vi "Ximea Camera Engine.vi"(0 "Ximea Notifier Name":string, 11 "Camera ID":string[](array[string])) -> ()   [LabVIEW 2016]
uses:
  Ximea Controls/Ximea ROI.ctl
  Ximea Controls/Ximea Parameters.ctl
  Ximea Controls/Ximea Parameter List.ctl
  xiLIB_64bit/xiLIB/xiCamLib/xiCam/PRM/PRM/PRM_v2.ctl
  Ximea Controls/Ximea Notifier Element.ctl
  Ximea Controls/Ximea Actions.ctl
  <vilib>/vision/Image Controls.llb/IMAQ Image.ctl
  Camera Controls/Camera IMAQ Key Info.ctl
panel:
  in  "Save Frames":bool
  in  "Use Display Module":bool
  in  "Quit":bool
  in  "Record":bool
  in  "Preview":bool
  out "Acquisition Loop":i32
  in  "Get Param":bool
  in  "Set Param":bool
  in  "Ximea  Parameter":T1
  in  "Get ROI":bool
  in  "Set ROI":bool
  in  "ROI Setup":T3
  out "Acquisition Frame":u32
  out "Serial No.":string
  out "Device Name":string
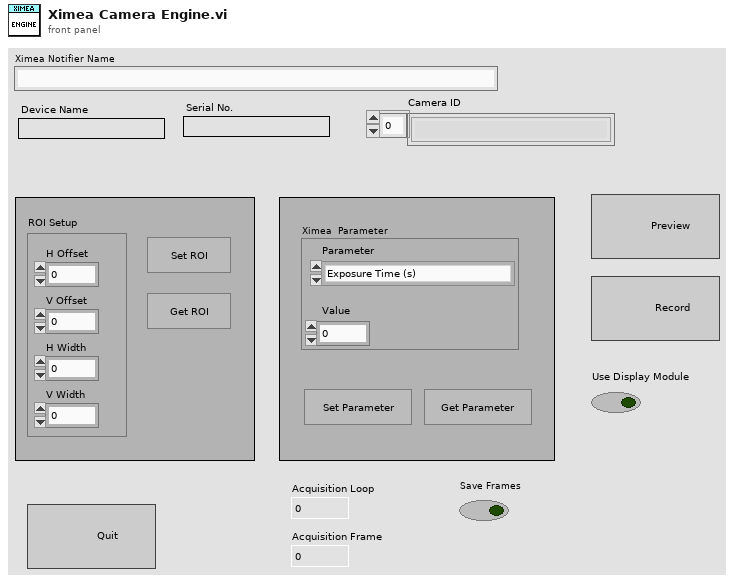
[diagram p1: front panel]
types:
  T1 = typedef "Ximea Parameters.ctl" = cluster{"Parameter":T2, "Value":sgl}
  T2 = typedef "Ximea Parameter List.ctl" = enum16{"Exposure Time (s)", "Gain"}
  T3 = typedef "Ximea ROI.ctl" = cluster{"H Offset":i32, "V Offset":i32, "H Width":i32, "V Width":i32}
  T4 = typedef "PRM_v2.ctl" = enum16{"ACQ_BUFFER_SIZE", "ACQ_FRAME_BURST_COUNT", "ACQ_TIMING_MODE", "ACQ_TRANSPORT_BUFFER_SIZE", "AE_MAX_LIMIT", "AEAG", "AEAG_LEVEL", "API_VERSION", "AG_MAX_LIMIT", "APPLY_CMS", "AUTO_BANDWIDTH_CALCULATION", "AUTO_WB", "AVAILABLE_BANDWIDTH", "AVAILABLE_BANDWIDTH_MAX", "AVAILABLE_BANDWIDTH_MIN", "BUFFER_POLICY", "BUFFERS_QUEUE_SIZE", "CC_MATRIX_00", "CC_MATRIX_01", "CC_MATRIX_02", "CC_MATRIX_03", "CC_MATRIX_10", "CC_MATRIX_11", "CC_MATRIX_12", "CC_MATRIX_13", "CC_MATRIX_20", "CC_MATRIX_21", "CC_MATRIX_22", "CC_MATRIX_23", "CC_MATRIX_30", "CC_MATRIX_31", "CC_MATRIX_32", "CC_MATRIX_33", "CHIP_TEMP", "CMS", "COLOR_FILTER_ARRAY", "COOLING", "DEBOUNCE_EN", "DEBOUNCE_POL", "DEBOUNCE_T0", "DEBOUNCE_T1", "DEBUG_LEVEL", "DEFAULT_CC_MATRIX", "DEVICE_INSTANCE_PATH", "DEVICE_MODEL_ID", "DEVICE_NAME", "DEVICE_SN", "DEVICE_TYPE", "DEVICE_USER_ID", "DOWNSAMPLING", "DOWNSAMPLING_TYPE", "DRV_VERSION", "EXP_PRIORITY", "EXPOSURE", "EXPOSURE_MAX", "EXPOSURE_MIN", "FFS_FILE_NAME", "FPGA1_VERSION", "FRAMERATE", "FRAMERATE_MAX", "FRAMERATE_MIN", "FREE_FFS_SIZE", "GAIN", "GAIN_MAX", "GAIN_MIN", "GAMMAC", "GAMMAY", "GPI_LEVEL", "GPI_MODE", "GPI_SELECTOR", "GPO_MODE", "GPO_SELECTOR", "HDR", "HDR_T1", "HDR_T2", "HEIGHT", "HEIGHT_MAX", "HEIGHT_MIN", "HOUSE_TEMP", "IMAGE_DATA_FORMAT", "IMAGE_IS_COLOR", "INPUT_CMS_PROFILE", "IS_COOLED", "IS_DEVICE_EXIST", "KNEEPOINT1", "KNEEPOINT2", "LED_MODE", "LED_SELECTOR", "LIMIT_BANDWIDTH", "LIMIT_BANDWIDTH_MAX", "LIMIT_BANDWIDTH_MIN", "LUT_EN", "LUT_INDEX", "LUT_INDEX_MAX", "LUT_INDEX_MIN", "LUT_VALUE", "LUT_VALUE_MAX", "LUT_VALUE_MIN", "MANUAL_WB", "MCU1_VERSION", "MCU2_VERSION", "OFFSET_X", "OFFSET_X_MAX", "OFFSET_X_MIN", "OFFSET_Y", "OFFSET_Y_MAX", "OFFSET_Y_MIN", "OUTPUT_CMS_PROFILE", "OUTPUT_DATA_BIT_DEPTH", "OUTPUT_DATA_PACKING", "READ_FILE_FFS", "RECENT_FRAME", "SENSOR_DATA_BIT_DEPTH", "SENSOR_MODE", "SENSOR_TAPS", "SHARPNESS", "SHUTTER_TYPE", "TARGET_TEMP", "TRG_DELAY", "TRG_SELECTOR", "TRG_SOFTWARE", "TRG_SOURCE", "USED_FFS_SIZE", "WB_KB", "WB_KG", "WB_KR", "WIDTH", "WIDTH_MAX", "WIDTH_MIN", "WRITE_FILE_FFS", "ACQ_BUFFER_SIZE_UNIT", "ACQ_TRANSPORT_BUFFER_COMMIT", "AEAG_ROI_HEIGHT", "AEAG_ROI_OFFSET_X", "AEAG_ROU_OFFSET_Y", "AEAG_ROI_WIDTH", "API_CONTEXT_LIST", "BINNING_HORIZONTAL", "BINNING_SELECTOR", "BINNING_VERTICAL", "COLUMN_FPN_CORRECTION", "COUNTER_SELECTOR", "COUNTER_VALUE", "DECIMATION_HORIZONTAL", "DECIMATION_SELECTOR", "DECIMATION_VERTICAL", "DEVICE_ID", "DEVICE_LOCATION_PATH", "DEVICE_MANIFEST", "DEVICE_RESET", "DEVICE_SENS_SN", "EXPOSURE_BURST_COUNT", "FFS_ACCESS_KEY", "GAIN_SELECTOR", "HW_REVISION", "IMAGE_BLACK_LEVEL", "IMAGE_DATA_BIT_DEPTH", "IMAGE_DATA_FORMAT_RGB32_ALPHA", "IMAGE_PAYLOAD_SIZE", "LENS_APERTURE_VALUE", "LENS_FEATURE", "LENS_FEATURE_SELECTOR", "LENS_FOCAL_LENGTH", "LENS_FOCUS_DISTANCE", "LENS_FOCUS_MOVE", "LENS_FOCUS_MOVEMENT_VALUE", "LENS_MODE", "OUTPUT_DATA_PACKING_TYPE", "SENSOR_CLOCK_FREQ_HZ", "SENSOR_CLOCK_FREQ_INDEX", "SENSOR_FEATURE_SELECTOR", "SENSOR_FEATURE_VALUE", "SENSOR_OUTPUT_CHANNEL_COUNT", "TRANSPORT_PIXEL_FORMAT", "TS_RST_MODE", "TS_RST_SOURCE", "SENS_DEFECTS_CORR_LIST_SELECTOR", "SENS_DEFECTS_CORR", "SENS_DEFECTS_CORR_LIST_CONTENT", "DEVICE_UNIT_SELECTOR", "DEVICE_UNIT_REGISTER_SELECTOR", "DEVICE_UNIT_REGISTER_VALUE"}
  T5 = typedef "Camera IMAQ Key Info.ctl" = cluster{"Frame":u32, "Sensor Height":i32, "Sensor Width":i32, "ROI Height":i32, "ROI Width":i32, "ROI Enable?":bool, "Bit per Pixel":u8}
  T6 = typedef "Image Type" = u32
  T7 = typedef "Ximea Notifier Element.ctl" = cluster{"Ximea Actions":T8, "Received?":bool, "Ximea Parameter":T1, "Ximea ROI":T3, "Running?":bool, "File Path":path, "# of frames":u32, "Image Ref":T9, "Error":errorcluster, "Trigger?":bool, "ROI Increment":i32}
  T8 = typedef "Ximea Actions.ctl" = enum16{"Idle", "Error Check", "Preview", "Record", "Soft Trigger", "Abort", "Record Settings", "Set Parameter", "Get Parameter", "Set ROI", "Get ROI", "Status", "Quit"}
  T9 = typedef "IMAQ Image.ctl" = refnum<image>
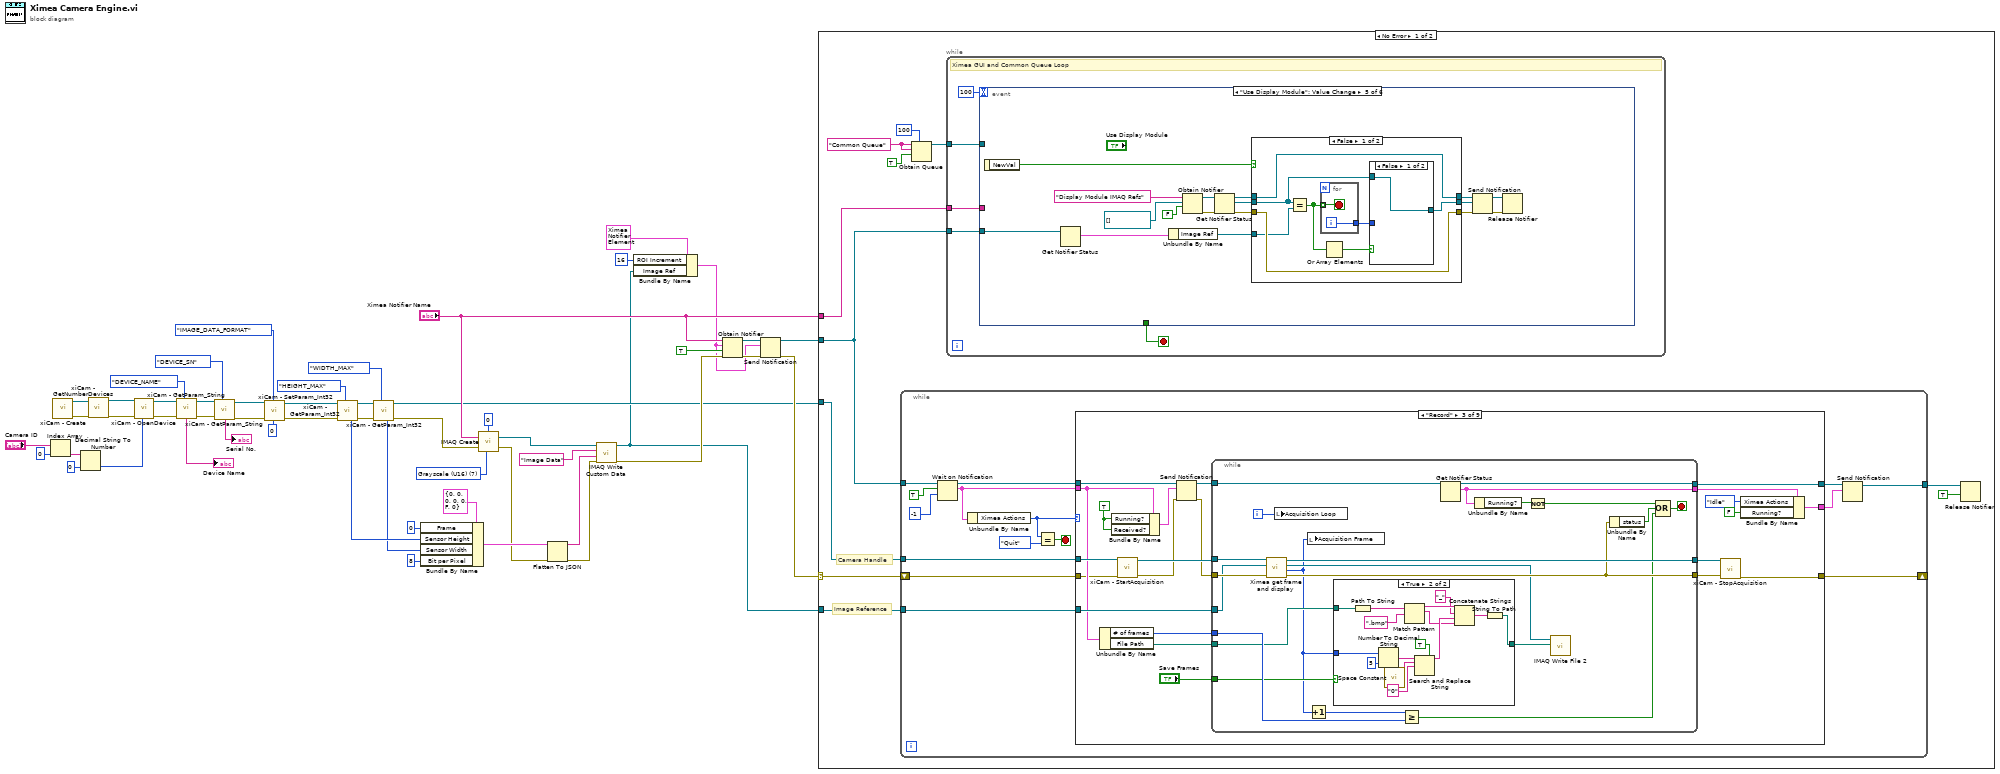
[diagram p0: block diagram]
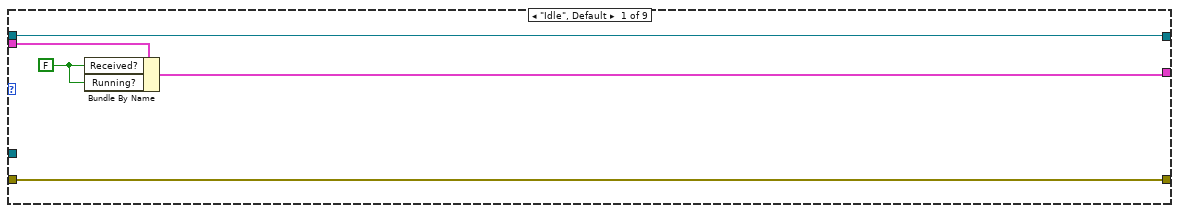
[diagram p2: hidden frame]
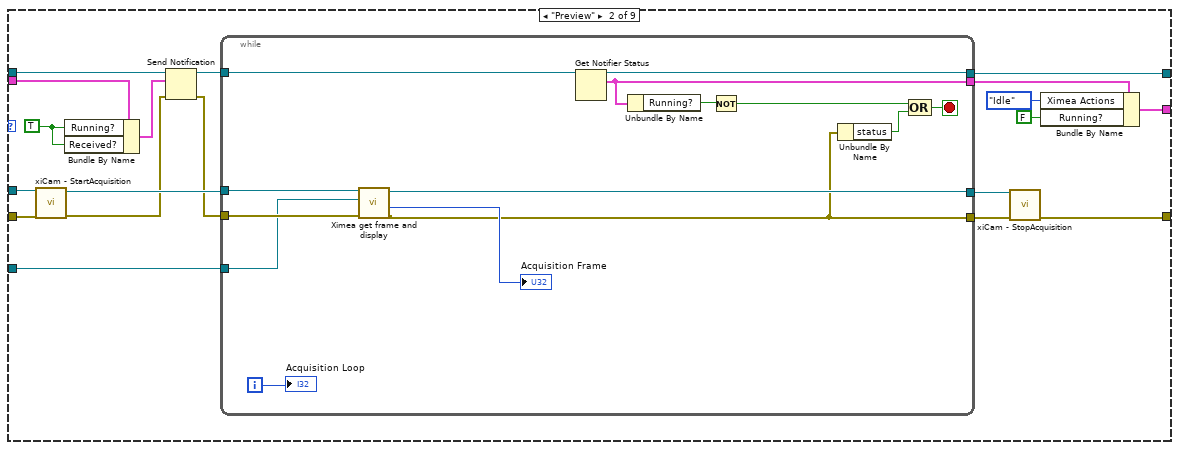
[diagram p3: hidden frame]
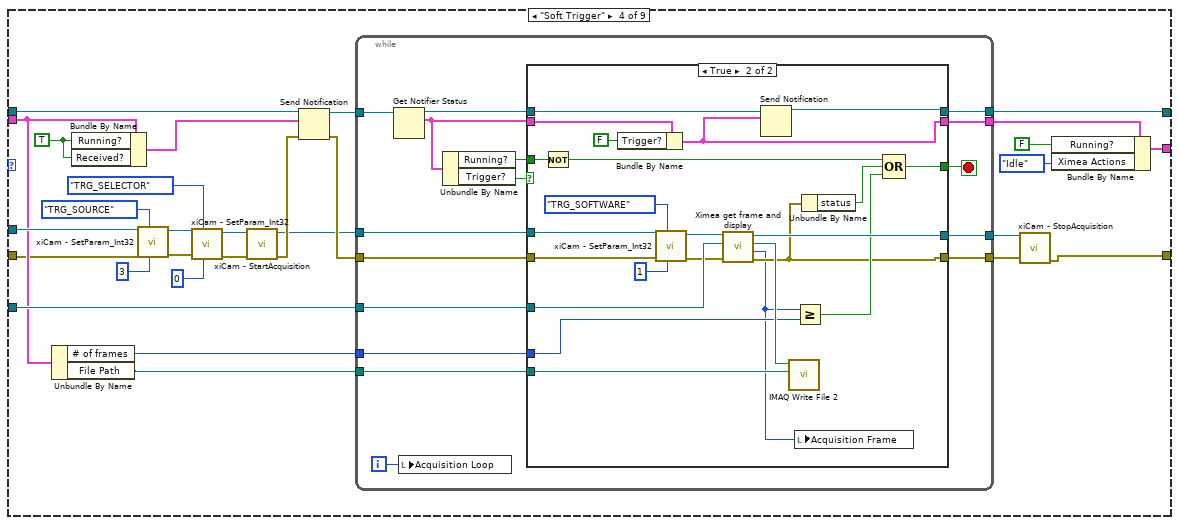
[diagram p5: hidden frame]
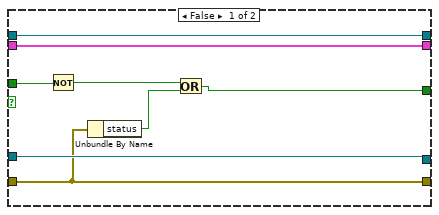
[diagram p6: hidden frame]
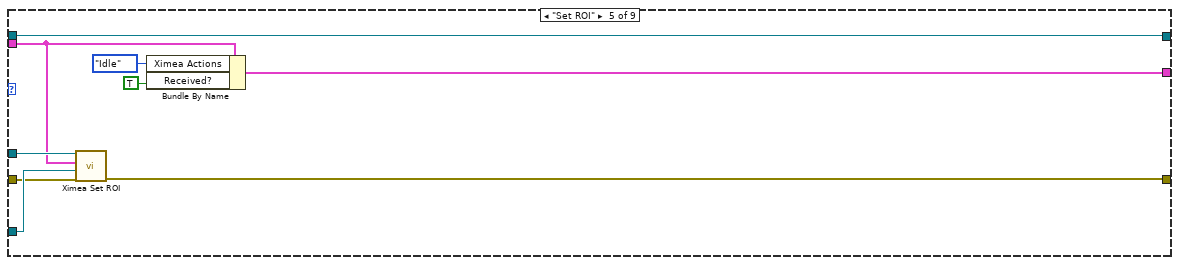
[diagram p7: hidden frame]
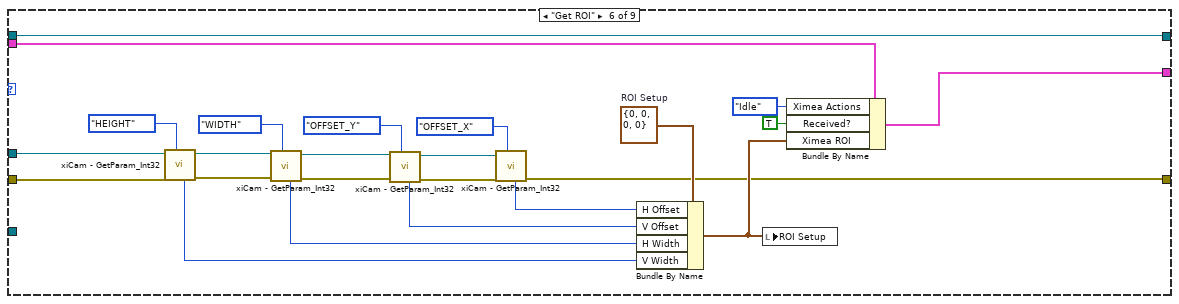
[diagram p8: hidden frame]
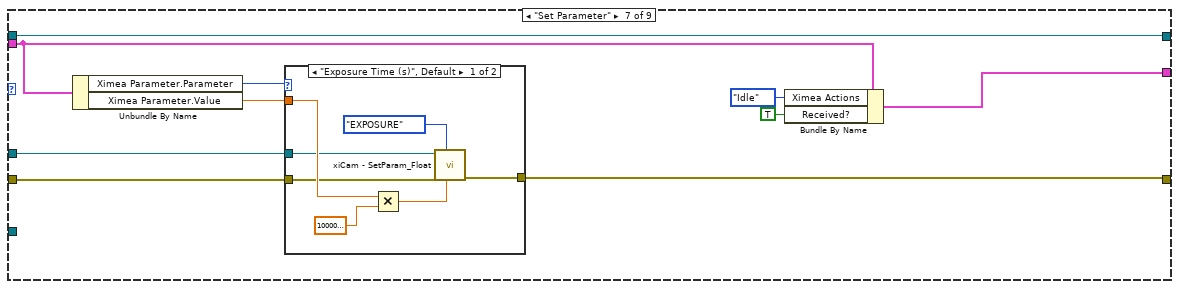
[diagram p9: hidden frame]
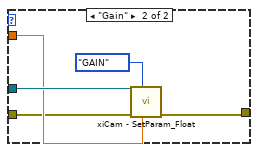
[diagram p10: hidden frame]
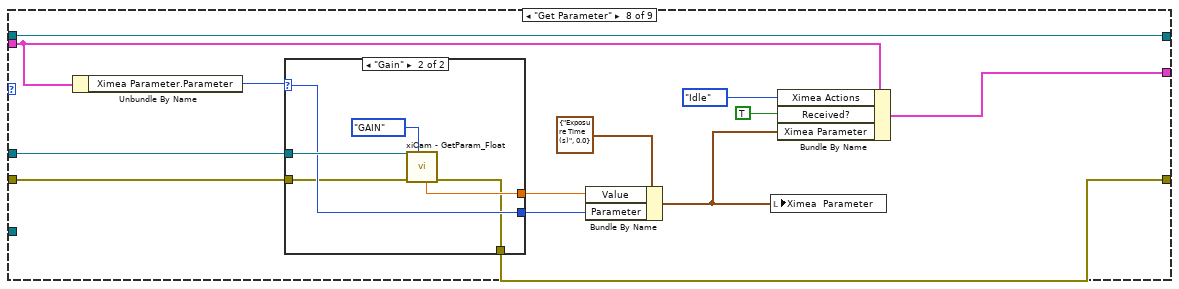
[diagram p11: hidden frame]
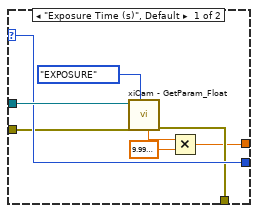
[diagram p12: hidden frame]
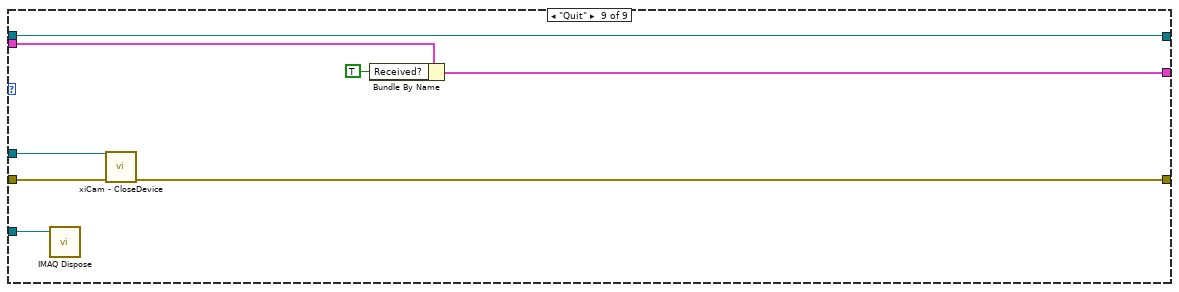
[diagram p13: hidden frame]
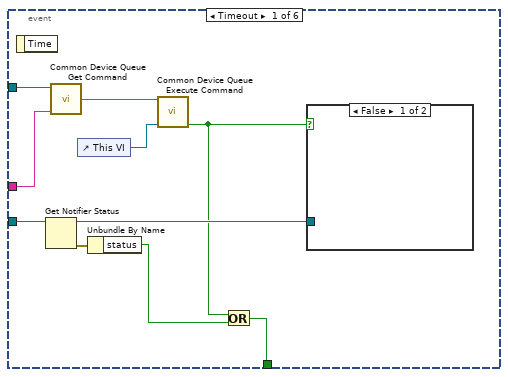
[diagram p14: hidden frame]
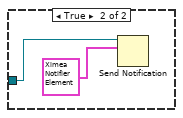
[diagram p15: hidden frame]
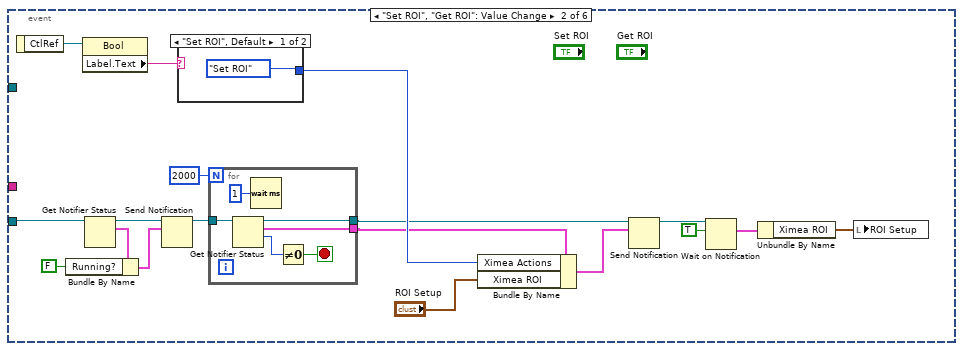
[diagram p16: hidden frame]
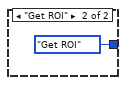
[diagram p17: hidden frame]
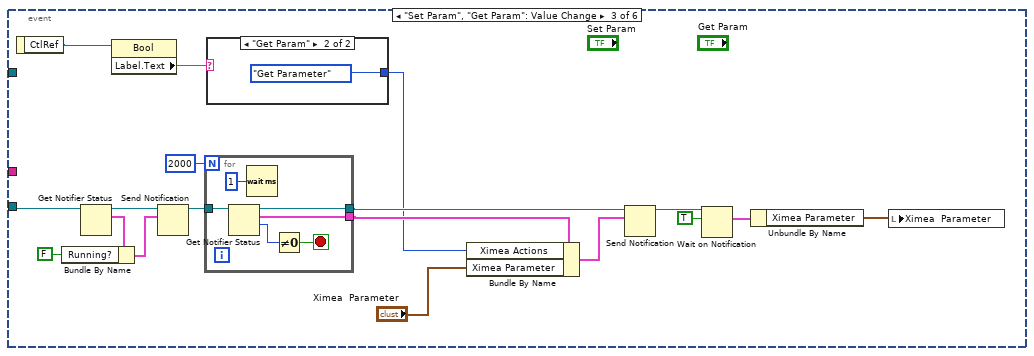
[diagram p18: hidden frame]
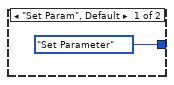
[diagram p19: hidden frame]
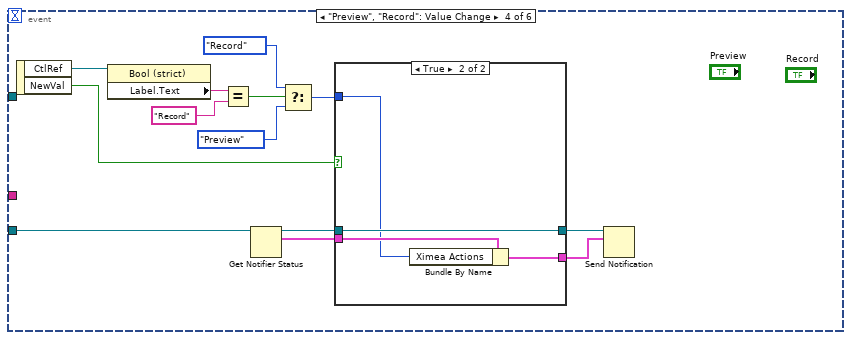
[diagram p20: hidden frame]
diagram:
  w35 = T6 7 items=["Grayscale (U8)", "Grayscale (I16)", "Grayscale (SGL)", "Complex (CSG)", "RGB (U32)", "HSL (U32)", "RGB (U64)", "Grayscale (U16)"] ("Image Type")
  n1 = Index Array(array="Camera ID", index=0) -> (element=w12:string)
  n2 = call "xiCam - Create.vi"() -> ("error out"=w51:errorcluster, "new xiCam"=w53:refnum<k24>)  [unwired: 10 in]
  n3 = Decimal String To Number(string=w12, default (0L)=u32 0 ("default (0 I32)")) -> (number=w10:u32)  [unwired: 1 in, 1 out]
  n4 = call "xiCam - GetNumberDevices.vi"("error in (no error)"=w51, "xiCam In"=w53) -> ("error out"=w50:errorcluster, "xiCam Out"=w52:refnum<k24>)  [unwired: 7 in, 1 out]
  n5 = call "xiCam - OpenDevice.vi"("DevID"=w10, "error in (no error)"=w50, "xiCam In"=w52) -> ("error out"=w22:errorcluster, "xiCam Out"=w30:refnum<k24>)  [unwired: 7 in]
  n6 = call "xiCam - GetParam_String.vi"("PRM"=PRM_v2."DEVICE_NAME", "error in (no error)"=w22, "xiCam In"=w30) -> ("error out"=w21:errorcluster, "xiCam Out"=w47:refnum<k24>, "String_Value"=→"Device Name":string)  [unwired: 6 in]
  n7 = call "xiCam - GetParam_String.vi"("PRM"=PRM_v2."DEVICE_SN", "error in (no error)"=w21, "xiCam In"=w47) -> ("error out"=w15:errorcluster, "xiCam Out"=w16:refnum<k24>, "String_Value"=→"Serial No.":string)  [unwired: 6 in]
  n8 = call "xiCam - SetParam_Int32.vi"("Int32_Value"=0, "PRM"=PRM_v2."IMAGE_DATA_FORMAT", "error in (no error)"=w15, "xiCam In"=w16) -> ("error out"=w9:errorcluster, "xiCam Out"=w8:refnum<k24>)  [unwired: 6 in]
  n9 = call "xiCam - GetParam_Int32.vi"("PRM"=PRM_v2."HEIGHT_MAX", "error in (no error)"=w9, "xiCam In"=w8) -> ("error out"=w6:errorcluster, "xiCam Out"=w7:refnum<k24>, "Int32_Value"=w31:i32)  [unwired: 6 in]
  n10 = call "xiCam - GetParam_Int32.vi"("PRM"=PRM_v2."WIDTH_MAX", "error in (no error)"=w6, "xiCam In"=w7) -> ("error out"=w5:errorcluster, "xiCam Out"=w4:refnum<k24>, "Int32_Value"=w28:i32)  [unwired: 6 in]
  n11 = Bundle By Name(cluster=T5 {"Frame"=0, "Sensor Height"=0, "Sensor Width"=0, "ROI Height"=0, "ROI Width"=0, "ROI Enable?"=FALSE, "Bit per Pixel"=0} ("Camera IMAQ Key Info"), "Frame"=u32 0, "Sensor Height"=w31, "Sensor Width"=w28, "Bit per Pixel"=u8 8) -> (w41:T5)
  n12 = call "IMAQ Create"("Border Size"=0, "Image Name"="Ximea Notifier Name", "Image Type"=w35, "error in (no error)"=w5) -> ("New Image"=w37:T9, "error out"=w34:errorcluster)  [unwired: 1 in]
  n13 = Flatten To JSON(anything=w41, error in (no error)=w34) -> (JSON string=w42:string, 11:w33:errorcluster)  [unwired: 1 in]
  n14 = call "IMAQ Write Custom Data"("error in (no error)"=w33, "Custom Data In"=w42, "Key"="Image Data", "Image"=w37) -> ("error out"=w26:errorcluster, "Image Out"=w2:T9)  [unwired: 6 in]
  n15 = Bundle By Name(cluster=T7 {"Ximea Actions"=enum."Error Check", "Received?"=FALSE, "Ximea Parameter"={"Parameter"=enum."Exposure Time (s)", "Value"=0.0}, "Ximea ROI"={"H Offset"=0, "V Offset"=0, "H Width"=0, "V Width"=0}, "Running?"=FALSE, "File Path"=path "", "# of frames"=0, "Image Ref"=refnum, "Error"={"status"=FALSE, "code"=0, "source"=""}, "Trigger?"=FALSE, "ROI Increment"=0} ("Ximea Camera Cluster"), "ROI Increment"=16, "Image Ref"=w2) -> (w3:T7)
  n16 = Obtain Notifier(name (unnamed)="Ximea Notifier Name", notification data type=w3, create if not found? (T)=TRUE, error in (no error)=w26) -> (notifier out=w44:refnum<notifier>, error out=w25:errorcluster)  [unwired: 1 out]
  n17 = Send Notification(notification=w3, notifier=w44, error in (no error)=w25) -> (notifier out=w24:refnum<notifier>, error out=w20:errorcluster)
  n18 = case shown="No Error" w20 {
    selector: w20 -> [w56 w481]
    tunnel: "Ximea Notifier Name" -> [w64 w483]
    tunnel: w24 -> [w59 w482]
    tunnel: w4 -> [w58 w479]
    tunnel: w2 -> [w57 w476]
    frame No Error {
      w63 = "Common Queue" ("Unique Notifier Name")
      # "Image Reference"
      # "Camera Handle"
      n19 = while {
        tunnel: w59 -> [w79]
        tunnel: w58 -> [w71]
        tunnel: w57 -> [w65]
        tunnel: [w68] -> w54
        shift-right: [w66] -> _
        shift-left: w56 -> [w67]
        stop <- w72 stop-if-true
        n20 = Wait on Notification(notifier=w79, ignore previous (F)=TRUE, timeout in ms (-1)=-1) -> (notifier out=w76:refnum<notifier>, notification=w75:T7)  [unwired: 1 in, 2 out]
        n21 = Unbundle By Name(w75) -> ("Ximea Actions"=w74:T8)
        n22 = Equal?(x=w74, y=Ximea_Actions."Quit") -> (x = y?=w72:bool)
        n23 = case shown="\"Record\"" w74 {
          tunnel: w76 -> [w82 w100 w136 w197 w261 w273 w292 w318 w339]
          tunnel: w75 -> [w84 w98 w123 w188 w256 w271 w291 w317 w338]
          tunnel: w71 -> [_ w102 w138 w203 w257 w281 w293 w319 w342]
          tunnel: w65 -> [_ w103 w139 w189 w255 _ _ _ w335]
          tunnel: [w82 w89 w126 w183 w261 w273 w292 w318 w339] -> w70
          tunnel: [w81 w88 w125 w181 w258 w267 w288 w314 w336] -> w69
          tunnel: w67 -> [w80 w85 w119 w177 w254 w266 w287 w309 w341]
          tunnel: [w80 w86 w120 w178 w253 w262 w286 w308 w340] -> w66
          frame "Idle", Default {
            w83 = FALSE ("Received?")
            n24 = Bundle By Name(cluster=w84, "Received?"=w83, "Running?"=w83) -> (w81:T7)
          }
          frame "Preview" {
            w97 = TRUE ("Received?")
            n25 = call "xiCam - StartAcquisition.vi"("error in (no error)"=w85, "xiCam In"=w102) -> ("error out"=w95:errorcluster, "xiCam Out"=w101:refnum<k24>)  [unwired: 8 in]
            n26 = Bundle By Name(cluster=w98, "Running?"=w97, "Received?"=w97) -> (w96:T7)
            n27 = Send Notification(notification=w96, notifier=w100, error in (no error)=w95) -> (notifier out=w99:refnum<notifier>, error out=w94:errorcluster)
            n28 = while {
              tunnel: w101 -> [w110]
              tunnel: w103 -> [w108]
              tunnel: w99 -> [w117]
              tunnel: w94 -> [w109]
              tunnel: [w116] -> w89
              tunnel: [w112] -> w91
              tunnel: [w106] -> w93
              tunnel: [w105] -> w92
              i -> [w104]
              stop <- w111 stop-if-true
              n29 = call "Ximea get frame and display.vi"("error in (no error)"=w109, "Image In"=w108, "xiCam In"=w110) -> ("error out"=w105:errorcluster, "FrameNumber"=→"Acquisition Frame":u32, "xiCam Out"=w106:refnum<k24>)  [unwired: 5 in, 1 out]
              n30 = Get Notifier Status(notifier=w117) -> (notifier out=w116:refnum<notifier>, current notification=w112:T7)  [unwired: 1 in, 3 out]
              n31 = Unbundle By Name(w112) -> ("Running?"=w115:bool)
              n32 = Not(x=w115) -> (.not. x?=w114:bool)
              n33 = Unbundle By Name(w105) -> ("status"=w113:bool)
              n34 = Compound Arithmetic op=OR(w114, w113) -> (w111:bool)
              "Acquisition Loop" <- w104
            }
            n35 = call "xiCam - StopAcquisition.vi"("error in (no error)"=w92, "xiCam In"=w93) -> ("error out"=w86:errorcluster)  [unwired: 8 in, 1 out]
            n36 = Bundle By Name(cluster=w91, "Ximea Actions"=Ximea_Actions."Idle", "Running?"=FALSE) -> (w88:T7)
          }
          frame "Record" {
            w134 = TRUE ("Received?")
            n37 = Unbundle By Name(w123) -> ("# of frames"=w122:u32, "File Path"=w121:path)
            n38 = Bundle By Name(cluster=w123, "Running?"=w134, "Received?"=w134) -> (w133:T7)
            n39 = call "xiCam - StartAcquisition.vi"("error in (no error)"=w119, "xiCam In"=w138) -> ("error out"=w132:errorcluster, "xiCam Out"=w137:refnum<k24>)  [unwired: 8 in]
            n40 = Send Notification(notification=w133, notifier=w136, error in (no error)=w132) -> (notifier out=w135:refnum<notifier>, error out=w131:errorcluster)
            n41 = while {
              tunnel: w137 -> [w160]
              tunnel: w139 -> [w158]
              tunnel: w135 -> [w157]
              tunnel: w131 -> [w159]
              tunnel: [w156] -> w126
              tunnel: [w152] -> w128
              tunnel: [w150] -> w130
              tunnel: [w149] -> w129
              tunnel: w122 -> [w147]
              tunnel: w121 -> [w144]
              tunnel: "Save Frames" -> [w142]
              i -> [w148]
              stop <- w151 stop-if-true
              n42 = call "Ximea get frame and display.vi"("error in (no error)"=w159, "Image In"=w158, "xiCam In"=w160) -> ("error out"=w149:errorcluster, "FrameNumber"=w141:u32, "Image Out"=w145:T9, "xiCam Out"=w150:refnum<k24>)  [unwired: 5 in]
              n43 = local write "Acquisition Loop"(w148) -> ()
              n44 = local write "Acquisition Frame"(w141) -> ()
              n45 = Increment(x=w141) -> (x+1=w140:u32)
              n46 = case shown="True" w142 {
                tunnel: w144 -> [w161 w176]
                tunnel: w141 -> [_ w167]
                tunnel: [w161 w162] -> w143
                frame False {
                }
                frame True {
                  n47 = Path To String(path=w176) -> (string=w175:string)
                  n48 = Number To Decimal String(number=w167, width (-)=i16 5) -> (decimal integer string=w171:string)
                  n49 = call <vilib>:"Space Constant.vi"() -> ("String"=w170:string)
                  n50 = Match Pattern(string=w175, regular expression=".bmp") -> (before substring=w173:string, match substring=w164:string)  [unwired: 1 in, 2 out]
                  n51 = Search and Replace String(replace all?=TRUE ("replace all? (F)"), input string=w171, search string=w170, replace string="0" ("replace string (\"\")")) -> (result string=w166:string)  [unwired: 4 in, 3 out]
                  n52 = Concatenate Strings(w173, "_" ("string"), w166, w164) -> (w163:string)
                  n53 = String To Path(string=w163) -> (path=w162:path)
                }
              }
              n54 = Greater Or Equal?(x=w140, y=w147) -> (x >= y?=w146:bool)
              n55 = Get Notifier Status(notifier=w157) -> (notifier out=w156:refnum<notifier>, current notification=w152:T7)  [unwired: 1 in, 3 out]
              n56 = Unbundle By Name(w152) -> ("Running?"=w155:bool)
              n57 = Not(x=w155) -> (.not. x?=w154:bool)
              n58 = call-poly "IMAQ Write File 2"("File Path"=w143, "Image"=w145) -> ()  [unwired: 8 in, 2 out]
              n59 = Unbundle By Name(w149) -> ("status"=w153:bool)
              n60 = Compound Arithmetic op=OR(w154, w153, w146) -> (w151:bool)
            }
            n61 = call "xiCam - StopAcquisition.vi"("error in (no error)"=w129, "xiCam In"=w130) -> ("error out"=w120:errorcluster)  [unwired: 8 in, 1 out]
            n62 = Bundle By Name(cluster=w128, "Ximea Actions"=Ximea_Actions."Idle", "Running?"=FALSE) -> (w125:T7)
          }
          frame "Soft Trigger" {
            w198 = TRUE ("Running?")
            n63 = Unbundle By Name(w188) -> ("# of frames"=w186:u32, "File Path"=w187:path)
            n64 = Bundle By Name(cluster=w188, "Running?"=w198, "Received?"=w198) -> (w196:T7)
            n65 = call "xiCam - SetParam_Int32.vi"("Int32_Value"=3, "PRM"=PRM_v2."TRG_SOURCE", "error in (no error)"=w177, "xiCam In"=w203) -> ("error out"=w195:errorcluster, "xiCam Out"=w202:refnum<k24>)  [unwired: 6 in]
            n66 = call "xiCam - SetParam_Int32.vi"("Int32_Value"=0, "PRM"=PRM_v2."TRG_SELECTOR", "error in (no error)"=w195, "xiCam In"=w202) -> ("error out"=w194:errorcluster, "xiCam Out"=w199:refnum<k24>)  [unwired: 6 in]
            n67 = call "xiCam - StartAcquisition.vi"("error in (no error)"=w194, "xiCam In"=w199) -> ("error out"=w193:errorcluster, "xiCam Out"=w190:refnum<k24>)  [unwired: 8 in]
            n68 = Send Notification(notification=w196, notifier=w197, error in (no error)=w193) -> (notifier out=w191:refnum<notifier>, error out=w192:errorcluster)
            n69 = while {
              tunnel: w192 -> [w217]
              tunnel: w191 -> [w221]
              tunnel: w190 -> [w219]
              tunnel: w189 -> [w218]
              tunnel: [w216] -> w185
              tunnel: w187 -> [w215]
              tunnel: w186 -> [w214]
              tunnel: [w210] -> w183
              tunnel: [w209] -> w182
              tunnel: [w208] -> w184
              i -> [w206]
              stop <- w207 stop-if-true
              n70 = Get Notifier Status(notifier=w221) -> (notifier out=w213:refnum<notifier>, current notification=w212:T7)  [unwired: 1 in, 3 out]
              n71 = local write "Acquisition Loop"(w206) -> ()
              n72 = Unbundle By Name(w212) -> ("Running?"=w211:bool, "Trigger?"=w220:bool)
              n73 = case shown="True" w220 {
                tunnel: w219 -> [w227 w252]
                tunnel: w218 -> [_ w248]
                tunnel: w217 -> [w224 w246]
                tunnel: [w227 w245] -> w216
                tunnel: w215 -> [_ w243]
                tunnel: w214 -> [_ w242]
                tunnel: w213 -> [w229 w238]
                tunnel: w212 -> [w228 w241]
                tunnel: w211 -> [w226 w239]
                tunnel: [w229 w237] -> w210
                tunnel: [w228 w232] -> w209
                tunnel: [w224 w231] -> w208
                tunnel: [w222 w233] -> w207
                frame False {
                  n74 = Not(x=w226) -> (.not. x?=w225:bool)
                  n75 = Unbundle By Name(w224) -> ("status"=w223:bool)
                  n76 = Or(x=w225, y=w223) -> (x .or. y?=w222:bool)
                }
                frame True {
                  n77 = Not(x=w239) -> (.not. x?=w236:bool)
                  n78 = Bundle By Name(cluster=w241, "Trigger?"=FALSE) -> (w232:T7)
                  n79 = call "xiCam - SetParam_Int32.vi"("Int32_Value"=1, "PRM"=PRM_v2."TRG_SOFTWARE", "error in (no error)"=w246, "xiCam In"=w252) -> ("error out"=w247:errorcluster, "xiCam Out"=w249:refnum<k24>)  [unwired: 6 in]
                  n80 = call "Ximea get frame and display.vi"("error in (no error)"=w247, "Image In"=w248, "xiCam In"=w249) -> ("error out"=w231:errorcluster, "FrameNumber"=w230:u32, "Image Out"=w244:T9, "xiCam Out"=w245:refnum<k24>)  [unwired: 5 in]
                  n81 = Send Notification(notification=w232, notifier=w238) -> (notifier out=w237:refnum<notifier>)  [unwired: 1 in, 1 out]
                  n82 = call-poly "IMAQ Write File 2"("File Path"=w243, "Image"=w244) -> ()  [unwired: 8 in, 2 out]
                  n83 = Greater Or Equal?(x=w230, y=w242) -> (x >= y?=w234:bool)
                  n84 = local write "Acquisition Frame"(w230) -> ()
                  n85 = Unbundle By Name(w231) -> ("status"=w235:bool)
                  n86 = Compound Arithmetic op=OR(w236, w235, w234) -> (w233:bool)
                }
              }
            }
            n87 = call "xiCam - StopAcquisition.vi"("error in (no error)"=w184, "xiCam In"=w185) -> ("error out"=w178:errorcluster)  [unwired: 8 in, 1 out]
            n88 = Bundle By Name(cluster=w182, "Running?"=FALSE, "Ximea Actions"=Ximea_Actions."Idle") -> (w181:T7)
          }
          frame "Set ROI" {
            n89 = call "Ximea Set ROI.vi"("error in"=w254, "Image Ref"=w255, "Ximea Camera Cluster"=w256, "xiCam In"=w257) -> ("error out"=w253:errorcluster)  [unwired: 6 in, 1 out]
            n90 = Bundle By Name(cluster=w256, "Ximea Actions"=Ximea_Actions."Idle", "Received?"=TRUE) -> (w258:T7)
          }
          frame "Get ROI" {
            w272 = T3 {"H Offset"=0, "V Offset"=0, "H Width"=0, "V Width"=0}  # ROI Setup
            n91 = call "xiCam - GetParam_Int32.vi"("PRM"=PRM_v2."HEIGHT", "error in (no error)"=w266, "xiCam In"=w281) -> ("error out"=w265:errorcluster, "xiCam Out"=w276:refnum<k24>, "Int32_Value"=w277:i32)  [unwired: 6 in]
            n92 = call "xiCam - GetParam_Int32.vi"("PRM"=PRM_v2."WIDTH", "error in (no error)"=w265, "xiCam In"=w276) -> ("error out"=w264:errorcluster, "xiCam Out"=w275:refnum<k24>, "Int32_Value"=w278:i32)  [unwired: 6 in]
            n93 = call "xiCam - GetParam_Int32.vi"("PRM"=PRM_v2."OFFSET_Y", "error in (no error)"=w264, "xiCam In"=w275) -> ("error out"=w263:errorcluster, "xiCam Out"=w274:refnum<k24>, "Int32_Value"=w279:i32)  [unwired: 6 in]
            n94 = call "xiCam - GetParam_Int32.vi"("PRM"=PRM_v2."OFFSET_X", "error in (no error)"=w263, "xiCam In"=w274) -> ("error out"=w262:errorcluster, "Int32_Value"=w280:i32)  [unwired: 6 in, 1 out]
            n95 = Bundle By Name(cluster=w272, "H Offset"=w280, "V Offset"=w279, "H Width"=w278, "V Width"=w277) -> (w270:T3)
            n96 = local write "ROI Setup"(w270) -> ()
            n97 = Bundle By Name(cluster=w271, "Ximea Actions"=Ximea_Actions."Idle", "Received?"=TRUE, "Ximea ROI"=w270) -> (w267:T7)
          }
          frame "Set Parameter" {
            n98 = Unbundle By Name(w291) -> ("Ximea Parameter.Parameter"=w295:T2, "Ximea Parameter.Value"=w294:sgl)
            n99 = case shown="\"Exposure Time (s)\", Default" w295 {
              tunnel: w294 -> [w301 w305]
              tunnel: w293 -> [w300 w307]
              tunnel: w287 -> [w297 w304]
              tunnel: [w296 w303] -> w286
              frame "Exposure Time (s)", Default {
                n100 = Multiply(x=w301, y=sgl 1000000.0) -> (x*y=w298:sgl)
                n101 = call "xiCam - SetParam_Float.vi"("Float_Value"=w298, "PRM"=PRM_v2."EXPOSURE", "error in (no error)"=w297, "xiCam In"=w300) -> ("error out"=w296:errorcluster)  [unwired: 6 in, 1 out]
              }
              frame "Gain" {
                n102 = call "xiCam - SetParam_Float.vi"("Float_Value"=w305, "PRM"=PRM_v2."GAIN", "error in (no error)"=w304, "xiCam In"=w307) -> ("error out"=w303:errorcluster)  [unwired: 6 in, 1 out]
              }
            }
            n103 = Bundle By Name(cluster=w291, "Ximea Actions"=Ximea_Actions."Idle", "Received?"=TRUE) -> (w288:T7)
          }
          frame "Get Parameter" {
            n104 = Unbundle By Name(w317) -> ("Ximea Parameter.Parameter"=w320:T2)
            n105 = case shown="\"Gain\"" w320 {
              selector: w320 -> [w326 w331]
              tunnel: w319 -> [w328 w334]
              tunnel: [w321 w332] -> w312
              tunnel: [w326 w331] -> w311
              tunnel: w309 -> [w325 w330]
              tunnel: [w324 w329] -> w308
              frame "Exposure Time (s)", Default {
                n106 = call "xiCam - GetParam_Float.vi"("PRM"=PRM_v2."EXPOSURE", "error in (no error)"=w325, "xiCam In"=w328) -> ("error out"=w324:errorcluster, "Float_Value"=w323:sgl)  [unwired: 6 in, 1 out]
                n107 = Multiply(x=w323, y=sgl 1e-06) -> (x*y=w321:sgl)
              }
              frame "Gain" {
                n108 = call "xiCam - GetParam_Float.vi"("PRM"=PRM_v2."GAIN", "error in (no error)"=w330, "xiCam In"=w334) -> ("error out"=w329:errorcluster, "Float_Value"=w332:sgl)  [unwired: 6 in, 1 out]
              }
            }
            n109 = Bundle By Name(cluster=T1 {"Parameter"=enum."Exposure Time (s)", "Value"=0.0} ("Ximea  Parameter"), "Value"=w312, "Parameter"=w311) -> (w310:T1)
            n110 = local write "Ximea  Parameter"(w310) -> ()
            n111 = Bundle By Name(cluster=w317, "Ximea Actions"=Ximea_Actions."Idle", "Received?"=TRUE, "Ximea Parameter"=w310) -> (w314:T7)
          }
          frame "Quit" {
            n112 = call "IMAQ Dispose"("Image"=w335) -> ()  [unwired: 5 in, 1 out]
            n113 = call "xiCam - CloseDevice.vi"("error in (no error)"=w341, "xiCam In"=w342) -> ("error out"=w340:errorcluster)  [unwired: 9 in]
            n114 = Bundle By Name(cluster=w338, "Received?"=TRUE) -> (w336:T7)
          }
        }
        n115 = Send Notification(notification=w69, notifier=w70) -> (notifier out=w68:refnum<notifier>)  [unwired: 1 in, 1 out]
      }
      n116 = Obtain Queue(max queue size (-1, unlimited)=100, name (unnamed)=w63, element data type=w63, create if not found? (T)=TRUE) -> (queue out=w60:refnum<queue>)  [unwired: 1 in, 2 out]
      n117 = while {
        tunnel: w64 -> [w346]
        tunnel: w60 -> [w345]
        tunnel: w59 -> [w344]
        stop <- w343 stop-if-true
        # "Ximea GUI and Common Queue Loop"
        n118 = event shown="[4] \"Use Display Module\": Value Change" {
          selector: _ -> [_ _ _ _ _ _]
          dyn-events: _ -> [_ _ _ _ _ _]
          timeout: 100 ("Numeric") -> [_ _ _ _ _ _]
          tunnel: w346 -> [w354 _ _ _ _ _]
          tunnel: w345 -> [w355 _ _ _ _ _]
          tunnel: w344 -> [w353 w366 w390 w416 w434 w473]
          tunnel: [w348 _ _ _ _ w475] -> w343
          event Timeout {
            n119 = event-data() -> ()  [unwired: 1 in, 1 out]
            n120 = Get Notifier Status(notifier=w353) -> (notifier out=w352:refnum<notifier>, error out=w351:errorcluster)  [unwired: 1 in, 3 out]
            n121 = call "Common Device Queue Get Command.vi"("Common Queue"=w355, "Notifier Name"=w354) -> ("Command"=w357:string)  [unwired: 12 in, 1 out]
            n122 = control-ref of="This VI"() -> (w356:refnum<vi>)
            n123 = Unbundle By Name(w351) -> ("status"=w349:bool)
            n124 = call "Common Device Queue Execute Command.vi"("Common Command"=w357, "VI Refnum"=w356) -> ("Quit?"=w350:bool)  [unwired: 12 in, 1 out]
            n125 = Or(x=w350, y=w349) -> (x .or. y?=w348:bool)
            n126 = case shown="False" w350 {
              tunnel: w352 -> [_ w359]
              frame False {
              }
              frame True {
                n127 = Send Notification(notification=T7 {"Ximea Actions"=enum."Error Check", "Received?"=FALSE, "Ximea Parameter"={"Parameter"=enum."Exposure Time (s)", "Value"=0.0}, "Ximea ROI"={"H Offset"=0, "V Offset"=0, "H Width"=0, "V Width"=0}, "Running?"=FALSE, "File Path"=path "", "# of frames"=0, "Image Ref"=refnum, "Error"={"status"=FALSE, "code"=0, "source"=""}, "Trigger?"=FALSE, "ROI Increment"=0} ("Ximea Camera Cluster"), notifier=w359) -> ()  [unwired: 1 in, 2 out]
              }
            }
          }
          event "Set ROI", "Get ROI": Value Change {
            n128 = event-data() -> ("CtlRef"=w377:refnum<vi>)  [unwired: 1 in]
            n129 = property class="Bool"(reference=w377) -> ("Label.Text"=w376:string)  [unwired: 1 in, 2 out]
            n130 = Get Notifier Status(notifier=w366) -> (notifier out=w369:refnum<notifier>, current notification=w372:T7)  [unwired: 1 in, 3 out]
            n131 = Bundle By Name(cluster=w372, "Running?"=FALSE) -> (w368:T7)
            n132 = Send Notification(notification=w368, notifier=w369) -> (notifier out=w367:refnum<notifier>)  [unwired: 1 in, 1 out]
            n133 = case shown="\"Set ROI\", Default" w376 {
              tunnel: [Ximea_Actions."Set ROI" ("Ximea Actions") Ximea_Actions."Get ROI" ("Ximea Actions")] -> w375
              frame "Set ROI", Default {
              }
              frame "Get ROI" {
              }
            }
            n134 = for {
              N: 2000 -> [_]
              tunnel: w367 -> [w382]
              tunnel: [w381] -> w365
              tunnel: [w380] -> w364
              stop <- w378 stop-if-true
              n135 = Get Notifier Status(notifier=w382) -> (notifier out=w381:refnum<notifier>, current notification=w380:T7, # waiting=w379:i32)  [unwired: 1 in, 2 out]
              n136 = Wait (ms)(milliseconds to wait=u32 1) -> ()  [unwired: 1 out]
              n137 = Not Equal To 0?(x=w379) -> (x != 0?=w378:bool)
            }
            n138 = Bundle By Name(cluster=w364, "Ximea Actions"=w375, "Ximea ROI"="ROI Setup") -> (w373:T7)
            n139 = Send Notification(notification=w373, notifier=w365) -> (notifier out=w363:refnum<notifier>)  [unwired: 1 in, 1 out]
            n140 = Wait on Notification(notifier=w363, ignore previous (F)=TRUE) -> (notification=w361:T7)  [unwired: 2 in, 3 out]
            n141 = Unbundle By Name(w361) -> ("Ximea ROI"=w360:T3)
            n142 = local write "ROI Setup"(w360) -> ()
          }
          event "Set Param", "Get Param": Value Change {
            n143 = event-data() -> ("CtlRef"=w402:refnum<vi>)  [unwired: 1 in]
            n144 = Get Notifier Status(notifier=w390) -> (notifier out=w397:refnum<notifier>, current notification=w400:T7)  [unwired: 1 in, 3 out]
            n145 = Bundle By Name(cluster=w400, "Running?"=FALSE) -> (w396:T7)
            n146 = property class="Bool"(reference=w402) -> ("Label.Text"=w403:string)  [unwired: 1 in, 2 out]
            n147 = Send Notification(notification=w396, notifier=w397) -> (notifier out=w395:refnum<notifier>)  [unwired: 1 in, 1 out]
            n148 = for {
              N: 2000 -> [_]
              tunnel: w395 -> [w408]
              tunnel: [w407] -> w394
              tunnel: [w406] -> w393
              stop <- w404 stop-if-true
              n149 = Get Notifier Status(notifier=w408) -> (notifier out=w407:refnum<notifier>, current notification=w406:T7, # waiting=w405:i32)  [unwired: 1 in, 2 out]
              n150 = Wait (ms)(milliseconds to wait=u32 1) -> ()  [unwired: 1 out]
              n151 = Not Equal To 0?(x=w405) -> (x != 0?=w404:bool)
            }
            n152 = case shown="\"Get Param\"" w403 {
              tunnel: [Ximea_Actions."Set Parameter" ("Ximea Actions") Ximea_Actions."Get Parameter" ("Ximea Actions")] -> w389
              frame "Set Param", Default {
              }
              frame "Get Param" {
              }
            }
            n153 = Bundle By Name(cluster=w393, "Ximea Actions"=w389, "Ximea Parameter"="Ximea  Parameter") -> (w401:T7)
            n154 = Send Notification(notification=w401, notifier=w394) -> (notifier out=w392:refnum<notifier>)  [unwired: 1 in, 1 out]
            n155 = Wait on Notification(notifier=w392, ignore previous (F)=TRUE) -> (notification=w387:T7)  [unwired: 2 in, 3 out]
            n156 = Unbundle By Name(w387) -> ("Ximea Parameter"=w386:T1)
            n157 = local write "Ximea  Parameter"(w386) -> ()
          }
          event "Preview", "Record": Value Change {
            n158 = event-data() -> ("CtlRef"=w424:refnum<vi>, "NewVal"=w418:bool)  [unwired: 1 in]
            n159 = property class="Bool (strict)"(reference=w424) -> ("Label.Text"=w423:string)  [unwired: 1 in, 2 out]
            n160 = Equal?(x=w423, y="Record") -> (x = y?=w421:bool)
            n161 = Get Notifier Status(notifier=w416) -> (notifier out=w415:refnum<notifier>, current notification=w414:T7)  [unwired: 1 in, 3 out]
            n162 = Select(t=Ximea_Actions."Record" ("Ximea Actions"), s=w421, f=Ximea_Actions."Preview") -> (s? t:f=w417:T8)
            n163 = case shown="True" w418 {
              tunnel: w417 -> [_ w430]
              tunnel: w415 -> [w428 w432]
              tunnel: w414 -> [w427 w431]
              tunnel: [w428 w432] -> w413
              tunnel: [w425 w429] -> w412
              frame False {
                n164 = Bundle By Name(cluster=w427, "Running?"=FALSE) -> (w425:T7)
              }
              frame True {
                n165 = Bundle By Name(cluster=w431, "Ximea Actions"=w430) -> (w429:T7)
              }
            }
            n166 = Send Notification(notification=w412, notifier=w413) -> ()  [unwired: 1 in, 2 out]
          }
          event "Use Display Module": Value Change {
            n167 = event-data() -> ("NewVal"=w433:bool)  [unwired: 1 in]
            n168 = Get Notifier Status(notifier=w434) -> (current notification=w449:T7)  [unwired: 1 in, 4 out]
            n169 = Unbundle By Name(w449) -> ("Image Ref"=w435:T9)
            n170 = Obtain Notifier(name (unnamed)="Display Module IMAQ Refs", notification data type=T9[] [], create if not found? (T)=FALSE) -> (notifier out=w442:refnum<notifier>, error out=w441:errorcluster)  [unwired: 1 in, 1 out]
            n171 = Get Notifier Status(notifier=w442, error in (no error)=w441) -> (notifier out=w443:refnum<notifier>, current notification=w445:T9[], error out=w444:errorcluster)  [unwired: 2 out]
            n172 = case shown="False" w433 {
              tunnel: w443 -> [w457 w467]
              tunnel: w444 -> [w451 w466]
              tunnel: w445 -> [w453 w469]
              tunnel: [w452 w468] -> w448
              tunnel: [w457 w467] -> w446
              tunnel: [w451 w466] -> w447
              tunnel: w435 -> [w450 w465]
              frame False {
                n173 = Equal?(x=w453, y=w450) -> (x = y?=w456:bool[])
                n174 = for {
                  tunnel: w456 -> [w464] mode=indexing
                  tunnel: [w463] -> w454
                  i -> [w463]
                  stop <- w464 stop-if-true
                }
                n175 = Or Array Elements(Boolean array=w456) -> (logical OR=w455:bool)
                n176 = case shown="False" w455 {
                  tunnel: w454 -> [_ w461]
                  tunnel: w453 -> [w458 w460]
                  tunnel: [w458 w459] -> w452
                  frame False {
                  }
                  frame True {
                    n177 = Delete From Array(array=w460, length=1, index=w461) -> (array with subset deleted=w459:T9[])  [unwired: 1 out]
                  }
                }
              }
              frame True {
                n178 = Build Array (concatenate)(w469, w465) -> (w468:T9[])
              }
            }
            n179 = Send Notification(notification=w448, notifier=w446, error in (no error)=w447) -> (notifier out=w440:refnum<notifier>, error out=w439:errorcluster)
            n180 = Release Notifier(notifier=w440, error in (no error)=w439) -> ()  [unwired: 1 in, 3 out]
          }
          event "Quit": Value Change {
            n181 = event-data() -> ("NewVal"=w475:bool)  [unwired: 1 in]
            n182 = Get Notifier Status(notifier=w473) -> (notifier out=w474:refnum<notifier>, current notification=w472:T7)  [unwired: 1 in, 3 out]
            n183 = Bundle By Name(cluster=w472, "Ximea Actions"=Ximea_Actions."Quit") -> (w471:T7)
            n184 = Send Notification(notification=w471, notifier=w474) -> ()  [unwired: 1 in, 2 out]
          }
        }
      }
      n185 = Release Notifier(notifier=w54, force destroy? (F)=TRUE) -> ()  [unwired: 1 in, 3 out]
    }
    frame Error {
      n186 = Release Notifier(notifier=w482, force destroy? (F)=TRUE, error in (no error)=w481) -> (error out=w480:errorcluster)  [unwired: 2 out]
      n187 = call "xiCam - CloseDevice.vi"("error in (no error)"=w480, "xiCam In"=w479) -> ("error out"=w478:errorcluster)  [unwired: 9 in]
      n188 = call "IMAQ Dispose"("Image"=w476, "error in (no error)"=w478) -> ("error out"=w477:errorcluster)  [unwired: 4 in]
      n189 = Unbundle By Name(w477) -> ("source"=w484:string)
      n190 = call <vilib>:"Space Constant.vi"() -> ("String"=w487:string)
      n191 = Concatenate Strings(w483, w487, "Device Error." ("string"), "\r", w484) -> (w488:string)
      n192 = One Button Dialog(message=w488) -> ()  [unwired: 1 in, 1 out]
    }
  }
